vi "P4_AbortVI.vi"(11 "Inputs":string[](array[string])) -> (2 "Output/Failure":string, 3 "CLI Process Return Code":i32)   [LabVIEW 2026]
doc: "Slice 1.1 probe: Open VI Reference, Run VI async, read state, Abort VI, read state, close the reference."
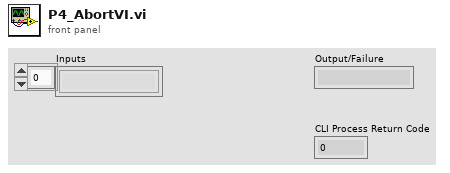
[diagram p1: front panel]
types:
  T1 = enum32{"Bad", "Idle", "Run top level", "Running"}
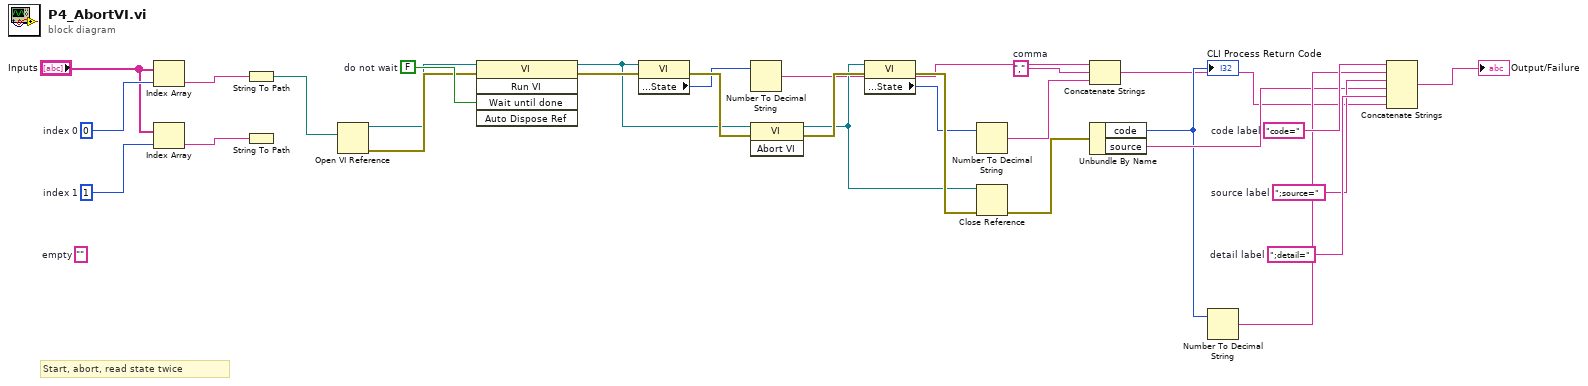
[diagram p0: block diagram]
diagram:
  w28 = ";detail="  # detail label
  w27 = ";source="  # source label
  w26 = "code="  # code label
  w20 = ","  # comma
  w9 = FALSE  # do not wait
  (unwired) ""  # empty
  w3 = 1  # index 1
  w2 = 0  # index 0
  # "Start, abort, read state twice"
  n1 = Index Array(array="Inputs", index=w2) -> (element=w4:string)
  n2 = Index Array(array="Inputs", index=w3) -> (element=w5:string)
  n3 = String To Path(string=w4) -> (path=w6:path)
  n4 = String To Path(string=w5) -> ()  [unwired: 1 out]
  n5 = Open VI Reference(vi path=w6) -> (vi reference=w7:refnum<vi>, error out=w8:errorcluster)  [unwired: 5 in]
  n6 = invoke class="VI" method="Run VI"(reference=w7, error in=w8, "Wait until done"=w9) -> (reference out=w10:refnum<vi>, error out=w11:errorcluster)  [unwired: 2 in, 3 out]
  n7 = property class="VI"(reference=w10, error in=w11) -> (error out=w13:errorcluster, "Execution:State"=w12:T1)  [unwired: 1 out]
  n8 = Number To Decimal String(number=w12) -> (decimal integer string=w14:string)  [unwired: 1 in]
  n9 = invoke class="VI" method="Abort VI"(reference=w10, error in=w13) -> (reference out=w15:refnum<vi>, error out=w16:errorcluster)  [unwired: 1 in, 1 out]
  n10 = property class="VI"(reference=w15, error in=w16) -> (error out=w18:errorcluster, "Execution:State"=w17:T1)  [unwired: 1 out]
  n11 = Number To Decimal String(number=w17) -> (decimal integer string=w19:string)  [unwired: 1 in]
  n12 = Close Reference(reference=w15, error in (no error)=w18) -> (error out=w22:errorcluster)
  n13 = Concatenate Strings(w14, w20, w19) -> (w21:string)
  n14 = Unbundle By Name(w22) -> ("code"=w23:i32, "source"=w24:string)
  "CLI Process Return Code" <- w23
  n15 = Number To Decimal String(number=w23) -> (decimal integer string=w25:string)  [unwired: 1 in]
  n16 = Concatenate Strings(w26, w25, w27, w24, w28, w21) -> (→"Output/Failure":string)
